vi "test_Mast Speed.vi"(8 "error in (no error)":errorcluster, 11 "TestCase in":refnum<class "CO3000 Test Case.lvclass">) -> (0 "error out":errorcluster, 3 "TestCase out":refnum<class "CO3000 Test Case.lvclass">)   [LabVIEW 2020, in "CO3000 Test Case.lvclass"]
uses:
  CO3000 Test Case.lvclass
  CO3000 Test Case.lvclass/CO3000 Test Case.ctl
  CO3000.lvclass/CO3000.ctl
  CO3000.lvclass
  <vilib>/addons/_JKI Toolkits/VI Tester/TestCase.llb/TestCase.lvclass
  C:/Program Files (x86)/National Instruments/LabVIEW 2020/vi.lib/addons/_JKI Toolkits/VI Tester/TestCase.llb/TestCase.lvclass
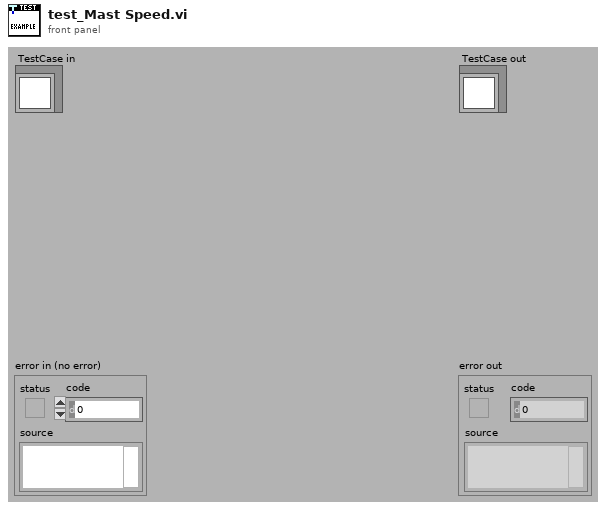
[diagram p1: front panel]
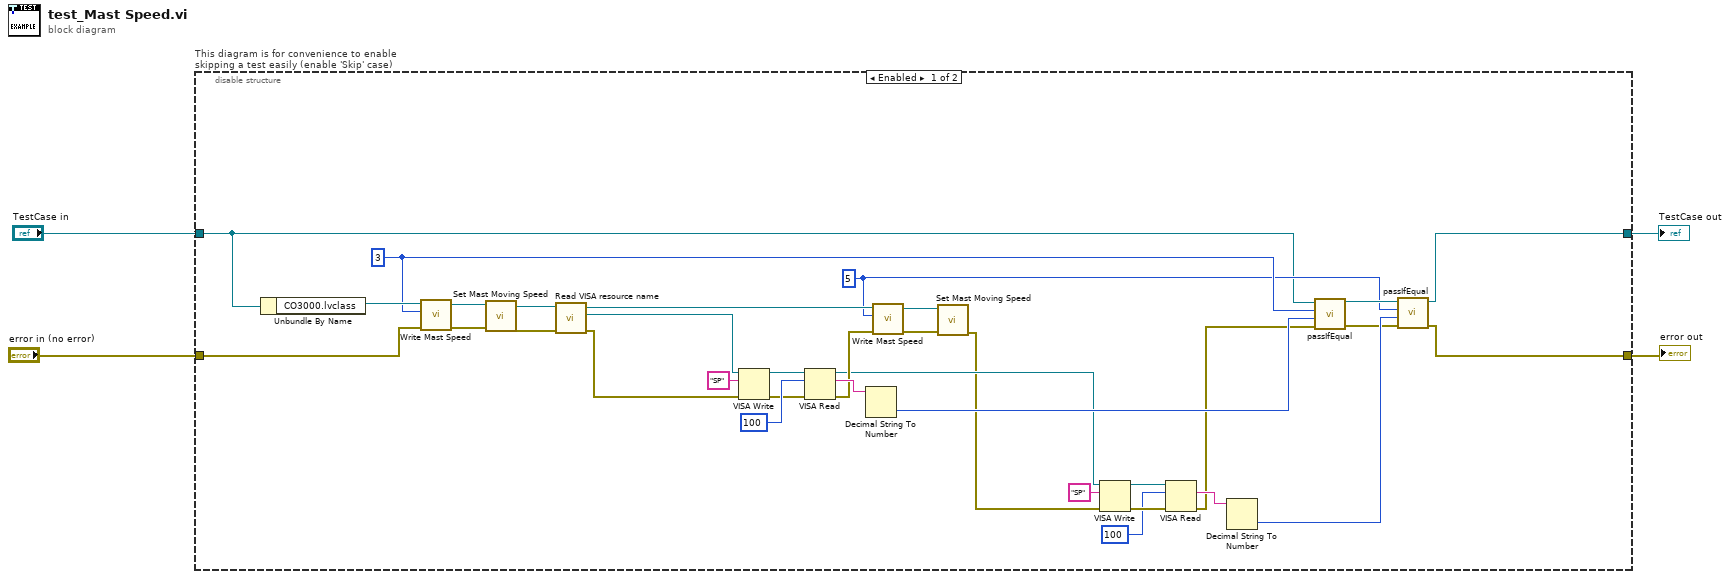
[diagram p0: block diagram]
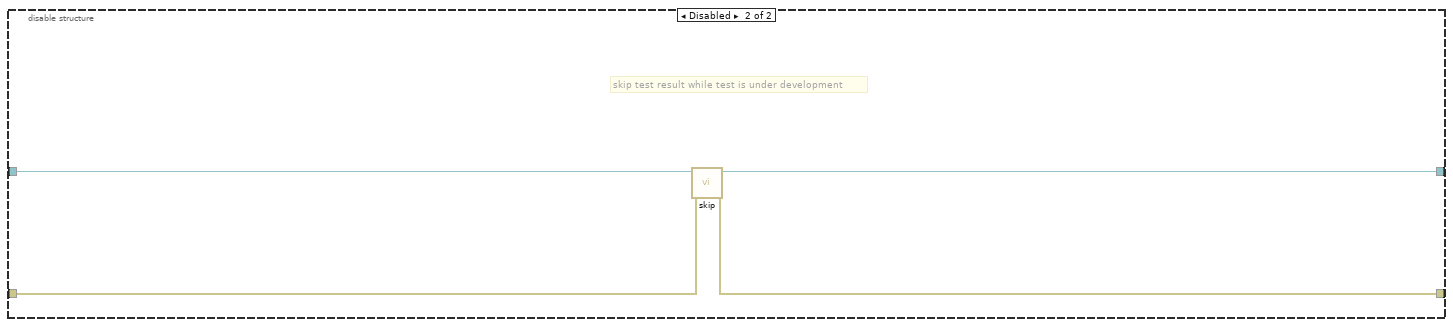
[diagram p2: hidden frame]
diagram:
  n1 = disable-structure "This diagram is for convenience to enable skipping a test easily (enable 'Skip' case)" shown="Enabled" {
    disable-tunnel: "TestCase in" -> [w5 w42]
    disable-tunnel: [w8 w40] -> w1
    disable-tunnel: [w7 w41] -> w3
    disable-tunnel: "error in (no error)" -> [w6 w39]
    frame Enabled {
      w12 = 5 ("Speed (1~8)")
      w35 = 3 ("Speed (1~8)")
      n2 = Unbundle By Name(w5) -> ("CO3000.lvclass"=w38:refnum<class "CO3000.lvclass">)
      n3 = call "Write Mast Speed.vi"("error in (no error)"=w6, "Speed (1~8)"=w35, "CO3000 in"=w38) -> ("error out"=w36:errorcluster, "CO3000 out"=w37:refnum<class "CO3000.lvclass">)  [unwired: 7 in]
      n4 = call-dynamic "Set Mast Moving Speed.vi"("error in (no error)"=w36, "CO3000 in"=w37) -> ("error out"=w33:errorcluster, "CO3000 out"=w34:refnum<class "CO3000.lvclass">)  [unwired: 8 in]
      n5 = call "Read VISA resource name.vi"("error in (no error)"=w33, "CO3000 in"=w34) -> ("error out"=w25:errorcluster, "VISA resource name"=w32:refnum<visa-resource-name>, "CO3000 out"=w22:refnum<class "CO3000.lvclass">)  [unwired: 7 in]
      n6 = VISA Write(VISA resource name=w32, write buffer="SP", error in (no error)=w25) -> (VISA resource name out=w30:refnum<visa-resource-name>, error out=w28:errorcluster)  [unwired: 1 out]
      n7 = VISA Read(VISA resource name=w30, byte count=u32 100, error in (no error)=w28) -> (VISA resource name out=w15:refnum<visa-resource-name>, read buffer=w27:string, error out=w21:errorcluster)  [unwired: 1 out]
      n8 = Decimal String To Number(string=w27) -> (number=w26:i32)  [unwired: 2 in, 1 out]
      n9 = call "Write Mast Speed.vi"("error in (no error)"=w21, "Speed (1~8)"=w12, "CO3000 in"=w22) -> ("error out"=w24:errorcluster, "CO3000 out"=w23:refnum<class "CO3000.lvclass">)  [unwired: 7 in]
      n10 = call-dynamic "Set Mast Moving Speed.vi"("error in (no error)"=w24, "CO3000 in"=w23) -> ("error out"=w14:errorcluster)  [unwired: 8 in, 1 out]
      n11 = VISA Write(VISA resource name=w15, write buffer="SP", error in (no error)=w14) -> (VISA resource name out=w17:refnum<visa-resource-name>, error out=w19:errorcluster)  [unwired: 1 out]
      n12 = VISA Read(VISA resource name=w17, byte count=u32 100, error in (no error)=w19) -> (read buffer=w20:string, error out=w10:errorcluster)  [unwired: 2 out]
      n13 = Decimal String To Number(string=w20) -> (number=w11:i32)  [unwired: 2 in, 1 out]
      n14 = call-dynamic "passIfEqual.vi"("error in (no error)"=w10, "y"=w26, "x"=w35, "TestCase in"=w5) -> ("error out"=w9:errorcluster, "TestCase out"=w13:refnum<class "CO3000 Test Case.lvclass">)  [unwired: 6 in]
      n15 = call-dynamic "passIfEqual.vi"("error in (no error)"=w9, "y"=w11, "x"=w12, "TestCase in"=w13) -> ("error out"=w7:errorcluster, "TestCase out"=w8:refnum<class "CO3000 Test Case.lvclass">)  [unwired: 6 in]
    }
    frame Disabled {
      # "skip test result while test is under development"
      n16 = call <vilib>:"skip.vi"("error in (no error)"=w39, "TestCase in"=w42) -> ("error out"=w41:errorcluster, "TestCase out"=w40:refnum<class "CO3000 Test Case.lvclass">)  [unwired: 8 in]
    }
  }
  "error out" <- w3
  "TestCase out" <- w1
